vi "setSerializedData.vi"(0 "reference":refnum<class "StateNode.lvclass">, 1 "parent":refnum<class "AbstractNode.lvclass">, 2 "children":refnum<class "AbstractNode.lvclass">[](array[class]), 3 "xmlOut":string, 5 "error in (no error)":errorcluster) -> (14 "reference out":refnum<class "StateNode.lvclass">, 19 "error out":errorcluster)   [LabVIEW 2020, in "StateNode.lvclass"]
doc: "setSerializedData"
uses:
  <resource>/Framework/Providers/Open_GDS/UML/StateNode_class/StateNode.lvclass
  C:/Program Files (x86)/National Instruments/LabVIEW 2020/resource/Framework/Providers/Open_GDS/UML/RectangularNode_class/RectangularNode.lvclass
  C:/Program Files (x86)/National Instruments/LabVIEW 2020/resource/Framework/Providers/Open_GDS/UML/AbstractNode_class/AbstractNode.lvclass
  <resource>/Framework/Providers/Open_GDS/UML/AbstractNode_class/AbstractNode.lvclass
  <resource>/Framework/Providers/Open_GDS/UML/General/Rectangle/Rectangle Rectangle2D.ctl
  <resource>/Framework/Providers/Open_GDS/UML/MultiLineString_class/MultiLineString.lvclass
  <resource>/Framework/Providers/Open_GDS/UML/RectangularNode_class/RectangularNode.lvclass
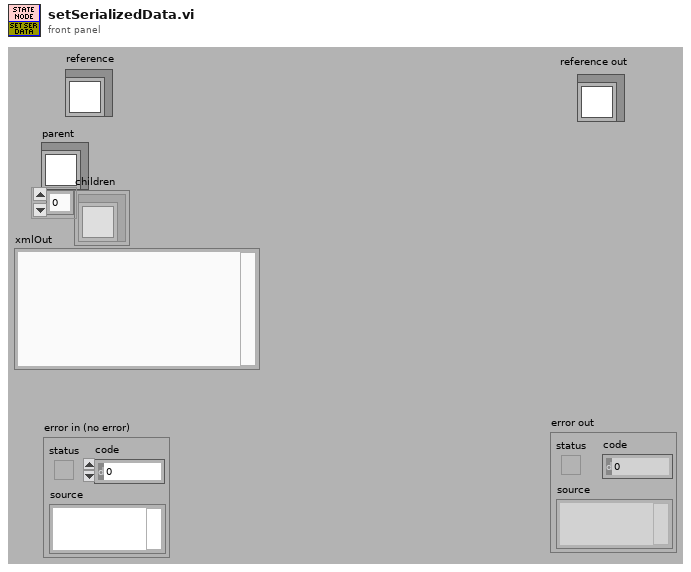
[diagram p1: front panel]
types:
  T1 = typedef "Rectangle Rectangle2D.ctl" = cluster{"x":dbl, "y":dbl, "width":dbl, "height":dbl}
  T2 = cluster{"Base class":cluster{"Base class":cluster{"parent":refnum<k1>, "children":refnum<k1>[]}, "bounds":T1}, "state":refnum<k1>, "action":refnum<k1>, "DEFAULT_WIDTH":i32, "DEFAULT_HEIGHT":i32}
  T3 = cluster{"Attributes":cluster{"Base class":cluster{"Base class":cluster{"parent":refnum<k1>, "children":refnum<k1>[]}, "bounds":T1}, "state":refnum<k1>, "action":refnum<k1>, "DEFAULT_WIDTH":i32, "DEFAULT_HEIGHT":i32}, string, string}
  T4 = typedef "RectangularNode.lvclass/ObjectAttributes.ctl" = cluster{"bounds":T1}
  T5 = typedef "AbstractNode.lvclass/ObjectAttributes.ctl" = cluster{"parent":refnum<class "AbstractNode.lvclass">, "children":refnum<class "AbstractNode.lvclass">[], "Hidden":bool}
  T6 = typedef "StateNode.lvclass/ObjectAttributes.ctl" = cluster{"state":refnum<class "MultiLineString.lvclass">, "action":refnum<class "MultiLineString.lvclass">, "DEFAULT_WIDTH":i32, "DEFAULT_HEIGHT":i32}
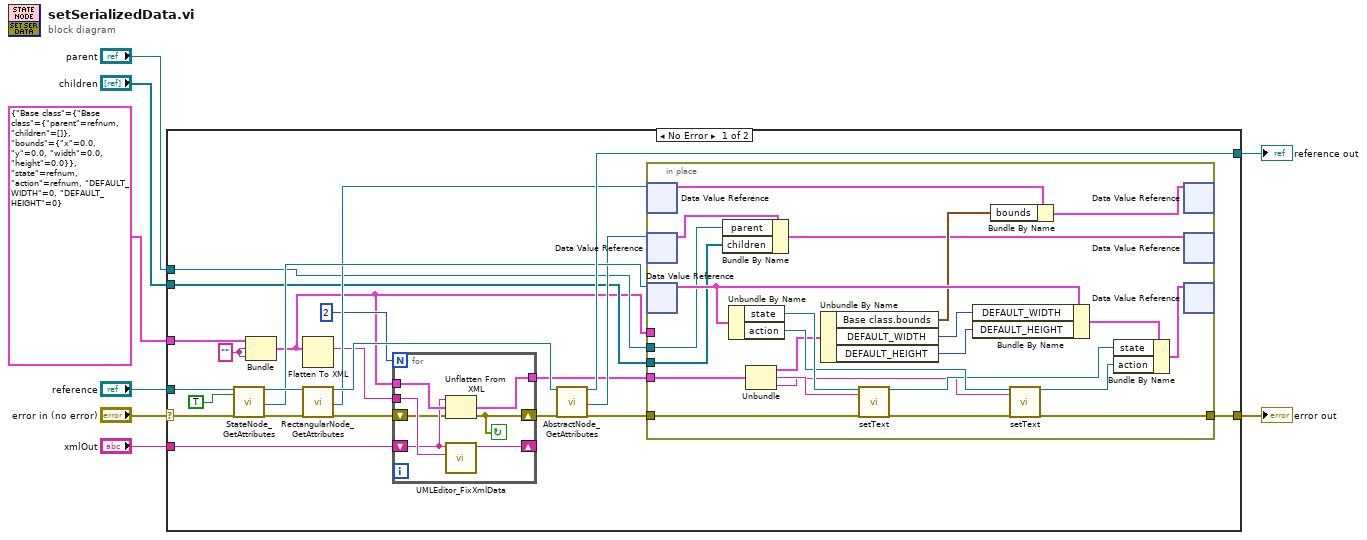
[diagram p0: block diagram]
diagram:
  n1 = case shown="No Error" "error in (no error)" {
    selector: "error in (no error)" -> [w30 w62]
    tunnel: "reference" -> [w31 w63]
    tunnel: [w29 w62] -> w6
    tunnel: [w28 w63] -> w5
    tunnel: "xmlOut" -> [w14 _]
    tunnel: "parent" -> [w17 _]
    tunnel: "children" -> [w16 _]
    tunnel: T2 {"Base class"={"Base class"={"parent"=refnum, "children"=[]}, "bounds"={"x"=0.0, "y"=0.0, "width"=0.0, "height"=0.0}}, "state"=refnum, "action"=refnum, "DEFAULT_WIDTH"=0, "DEFAULT_HEIGHT"=0} ("Attributes") -> [w26 _]
    frame No Error {
      w27 = ""
      n2 = call <resource>:"StateNode_GetAttributes.vi"("reference in"=w31, "OnlyGetDvrReference(False)"=TRUE, "error in (no error)"=w30) -> ("reference out"=w24:refnum<class "StateNode.lvclass">, "DataRef"=w21:refnum<data-value>, "error out"=w23:errorcluster)  [unwired: 13 in, 1 out]
      n3 = Bundle("Attributes"=w26, w27, w27) -> (w13:T3)  [unwired: 1 out]
      n4 = Flatten To XML(6:w13) -> (2:w12:string)
      n5 = call <resource>:"RectangularNode_GetAttributes.vi"("reference in"=w24, "error in (no error)"=w23) -> ("reference out"=w22:refnum<class "StateNode.lvclass">, "DataRef"=w20:refnum<data-value>, "error out"=w10:errorcluster)  [unwired: 14 in, 1 out]
      n6 = for {
        N: 2 -> [_]
        tunnel: [w38] -> w11
        tunnel: w12 -> [w37]
        tunnel: w13 -> [w36]
        shift-right: [w34] -> _
        shift-left: w14 -> [w33]
        shift-right: [w35] -> w9
        shift-left: w10 -> [w32]
        stop <- w35 continue-if-true
        n7 = Unflatten From XML(xml string=w33, type=w36, error in (no error)=w32) -> (value=w38:T3, error out=w35:errorcluster)
        n8 = call <resource>:"UMLEditor_FixXmlData.vi"("XmlTemplateIn"=w37, "xmlIn"=w33) -> ("XML OUt"=w34:string)  [unwired: 9 in]
      }
      n9 = call <resource>:"AbstractNode_GetAttributes.vi"("reference in"=w22, "error in (no error)"=w9) -> ("reference out"=w28:refnum<class "StateNode.lvclass">, "DataRef"=w19:refnum<data-value>, "error out"=w18:errorcluster)  [unwired: 14 in, 1 out]
      n10 = in-place {
        in-place-border: [w47] -> w29
        in-place-border: w18 -> [w39]
        in-place-border: w13 -> [_]
        in-place-border: w17 -> [w43]
        in-place-border: w16 -> [w42]
        in-place-border: w11 -> [w40]
        n11 = in-place-dvr #1(w20) -> (w46:T4)  [unwired: 1 out]
        n12 = in-place-dvr #2(w19) -> (w44:T5)  [unwired: 1 out]
        n13 = in-place-dvr #3(w21) -> (w61:T6)  [unwired: 1 out]
        n14 = Bundle By Name(cluster=w44, "parent"=w43, "children"=w42) -> (w41:T5)
        n15 = Unbundle By Name(w61) -> ("state"=w57:refnum<class "MultiLineString.lvclass">, "action"=w56:refnum<class "MultiLineString.lvclass">)
        n16 = Unbundle(w40) -> ("Attributes"=w52:T2, w50:string, w48:string)
        n17 = Unbundle By Name(w52) -> ("Base class.bounds"=w51:T1, "DEFAULT_WIDTH"=w60:i32, "DEFAULT_HEIGHT"=w59:i32)
        n18 = call-dynamic "setText.vi"("reference"=w57, "text"=w50, "error in (no error)"=w39) -> ("reference out"=w55:refnum<class "MultiLineString.lvclass">, "error out"=w49:errorcluster)  [unwired: 15 out]
        n19 = Bundle By Name(cluster=w61, "DEFAULT_WIDTH"=w60, "DEFAULT_HEIGHT"=w59) -> (w58:T6)
        n20 = Bundle By Name(cluster=w46, "bounds"=w51) -> (w45:T4)
        n21 = call-dynamic "setText.vi"("reference"=w56, "text"=w48, "error in (no error)"=w49) -> ("reference out"=w54:refnum<class "MultiLineString.lvclass">, "error out"=w47:errorcluster)  [unwired: 15 out]
        n22 = Bundle By Name(cluster=w58, "state"=w55, "action"=w54) -> (w53:T6)
        n23 = in-place-dvr #1(w45) -> ()  [unwired: 2 out]
        n24 = in-place-dvr #2(w41) -> ()  [unwired: 2 out]
        n25 = in-place-dvr #3(w53) -> ()  [unwired: 2 out]
      }
    }
    frame Error {
    }
  }
  "reference out" <- w5
  "error out" <- w6
